vi "GUI_Bella_IP2_plasma1.vi"() -> ()   [LabVIEW 2020]
uses:
  Shared/GUI_Template/GUI_master/tcp_new_data_event.ctl
  Shared/GUI_Template/GUI_master/tcp new data cluster.ctl
panel:
  in  "Position.Axis 2::9":dbl caption="1: Ghost z-position" min=0.0 max=100.0 format="%.3g"
  in  "Position.Axis 1::9":dbl caption="1: Staging Sideview" min=-50.0 max=50.0 format="%.3g"
  in  "GUIdevice 9":string="MCD-PL1-ESP301-1" caption="GUIdevice 4"
  in  "Position.Stage B::19":dbl caption="DPM - Y" min=-100.0 max=105.0 format="%.3g"
  in  "Position.Stage C::18":dbl caption="DPM - Z" min=-100.0 max=100.0 format="%.3g"
  in  "Position.Stage A::18":dbl caption="DPM - X" min=-400.0 max=400.0 format="%.3g"
  in  "GUIdevice 19":string="MCD-PL1-NewmarkDPMY"
  in  "GUIdevice 18":string="MCD-PL1-NewmarkDPMXZ"
  in  "GUIdevice 17":string="IP2-TargetXYZ"
  in  "Position.Axis 1::17":dbl caption="TargetX" min=-200.0 max=200.0 format="%.3g"
  in  "Position.Axis 2::17":dbl caption="Peptide Stage" min=-200.0 max=150.0 format="%.3g"
  in  "Position.Axis 3::17":dbl caption="TargetZ" min=-100.0 max=50.0 format="%.3g"
  in  "GUIdevice 16":string="IP2-TC-ESP5"
  in  "Position.Axis 1::16":dbl caption="Quad 1-2 \n[In = 0, Out = -45]" min=-50.0 max=50.0 format="%.3g"
  in  "Position.Axis 2::16":dbl caption="Quad 3\n[In = 0, Out = 74]" min=-100.0 max=100.0 format="%.3g"
  in  "Position.Axis 3::16":dbl caption="Quad 4 \n[In = 0, Out = 80]" min=-100.0 max=100.0 format="%.3g"
  in  "GUIdevice 15":string="IP2-TC-ESP5"
  in  "Position.Axis 1::15":dbl caption="OPEN" min=-50.0 max=50.0 format="%.3g"
  in  "Position.Axis 2::15":dbl caption="OPEN" min=-100.0 max=100.0 format="%.3g"
  in  "Position.Axis 3::15":dbl caption="OPEN" min=-100.0 max=100.0 format="%.3g"
  in  "GUIdevice 14":string="IP2-TC-ESP3"
  in  "Position.Axis 1::14":dbl caption="TapeDrive Z" min=-25.0 max=25.0 format="%.3g"
  in  "Position.Axis 2::14":dbl caption="IP2-focusdiag-x" min=-25.0 max=25.0 format="%.3g"
  in  "Position.Axis 3::14":dbl caption="Target scatter lens" min=0.0 max=25.0 format="%.3g"
  in  "GUIdevice 13":string="IP2-TC-ESP4"
  in  "Position.Axis 1::13":dbl caption="OAPT-Horz (Yaw)" min=-3.0 max=9.0 format="%.3g"
  in  "Position.Axis 2::13":dbl caption="OAPT-Vert (Pitch)" min=-3.0 max=3.0 format="%.3g"
  in  "Position.Axis 3::13":dbl caption="Profiler Block" min=0.0 max=100.0 format="%.3g"
  in  "GUIdevice 12":string="IP2-BTL-ESP2"
  in  "Position.Axis 1::12":dbl caption="IP2 M5 vrt" min=0.0 max=20.0 format="%.3g"
  in  "Position.Axis 2::12":dbl caption="IP2 M6 (SFL) vrt" min=-20.0 max=20.0 format="%.3g"
  in  "Position.Axis 3::12":dbl caption="IP2 M3 (LFL) vrt" min=-20.0 max=20.0 format="%.3g"
  in  "Position.Axis 3::11":dbl caption="IP2 M3 (LFL) hrz" min=-20.0 max=20.0 format="%.3g"
  in  "Position.Axis 2::11":dbl caption="IP2 M6 (SFL) hrz" min=0.0 max=20.0 format="%.3g"
  in  "Position.Axis 1::11":dbl caption="IP2 M5 hrz" min=-20.0 max=20.0 format="%.3g"
  in  "GUIdevice 11":string="IP2-BTL-ESP1"
  in  "GUIdevice 10":string="IP2-TC-ESP3"
  in  "Position.Axis 2::10":dbl caption="Focus diag X" min=-25.0 max=25.0 format="%.3g"
  in  "Position.Axis 3::8":dbl caption="Focus diag Z" min=-5.0 max=100.0 format="%.3g"
  in  "Position.Axis 2::8":dbl caption="Focus diag Y" min=-5.0 max=150.0 format="%.3g"
  in  "GUIdevice 8":string="IP2-focusdiag-zy" caption="GUIdevice 4"
  out "tcp data event":T1
  in  "stop":bool
  out "error IO 2":errorcluster
  # "Plasma 1 + M Chambers"
  # "TC-ESP3"
  # "TC-ESP4"
  # "TC-ESP5"
  # "TC-ESP6"
  # "Target-XYZ"
  # "BTL-ESP1"
  # "BTL-ESP2"
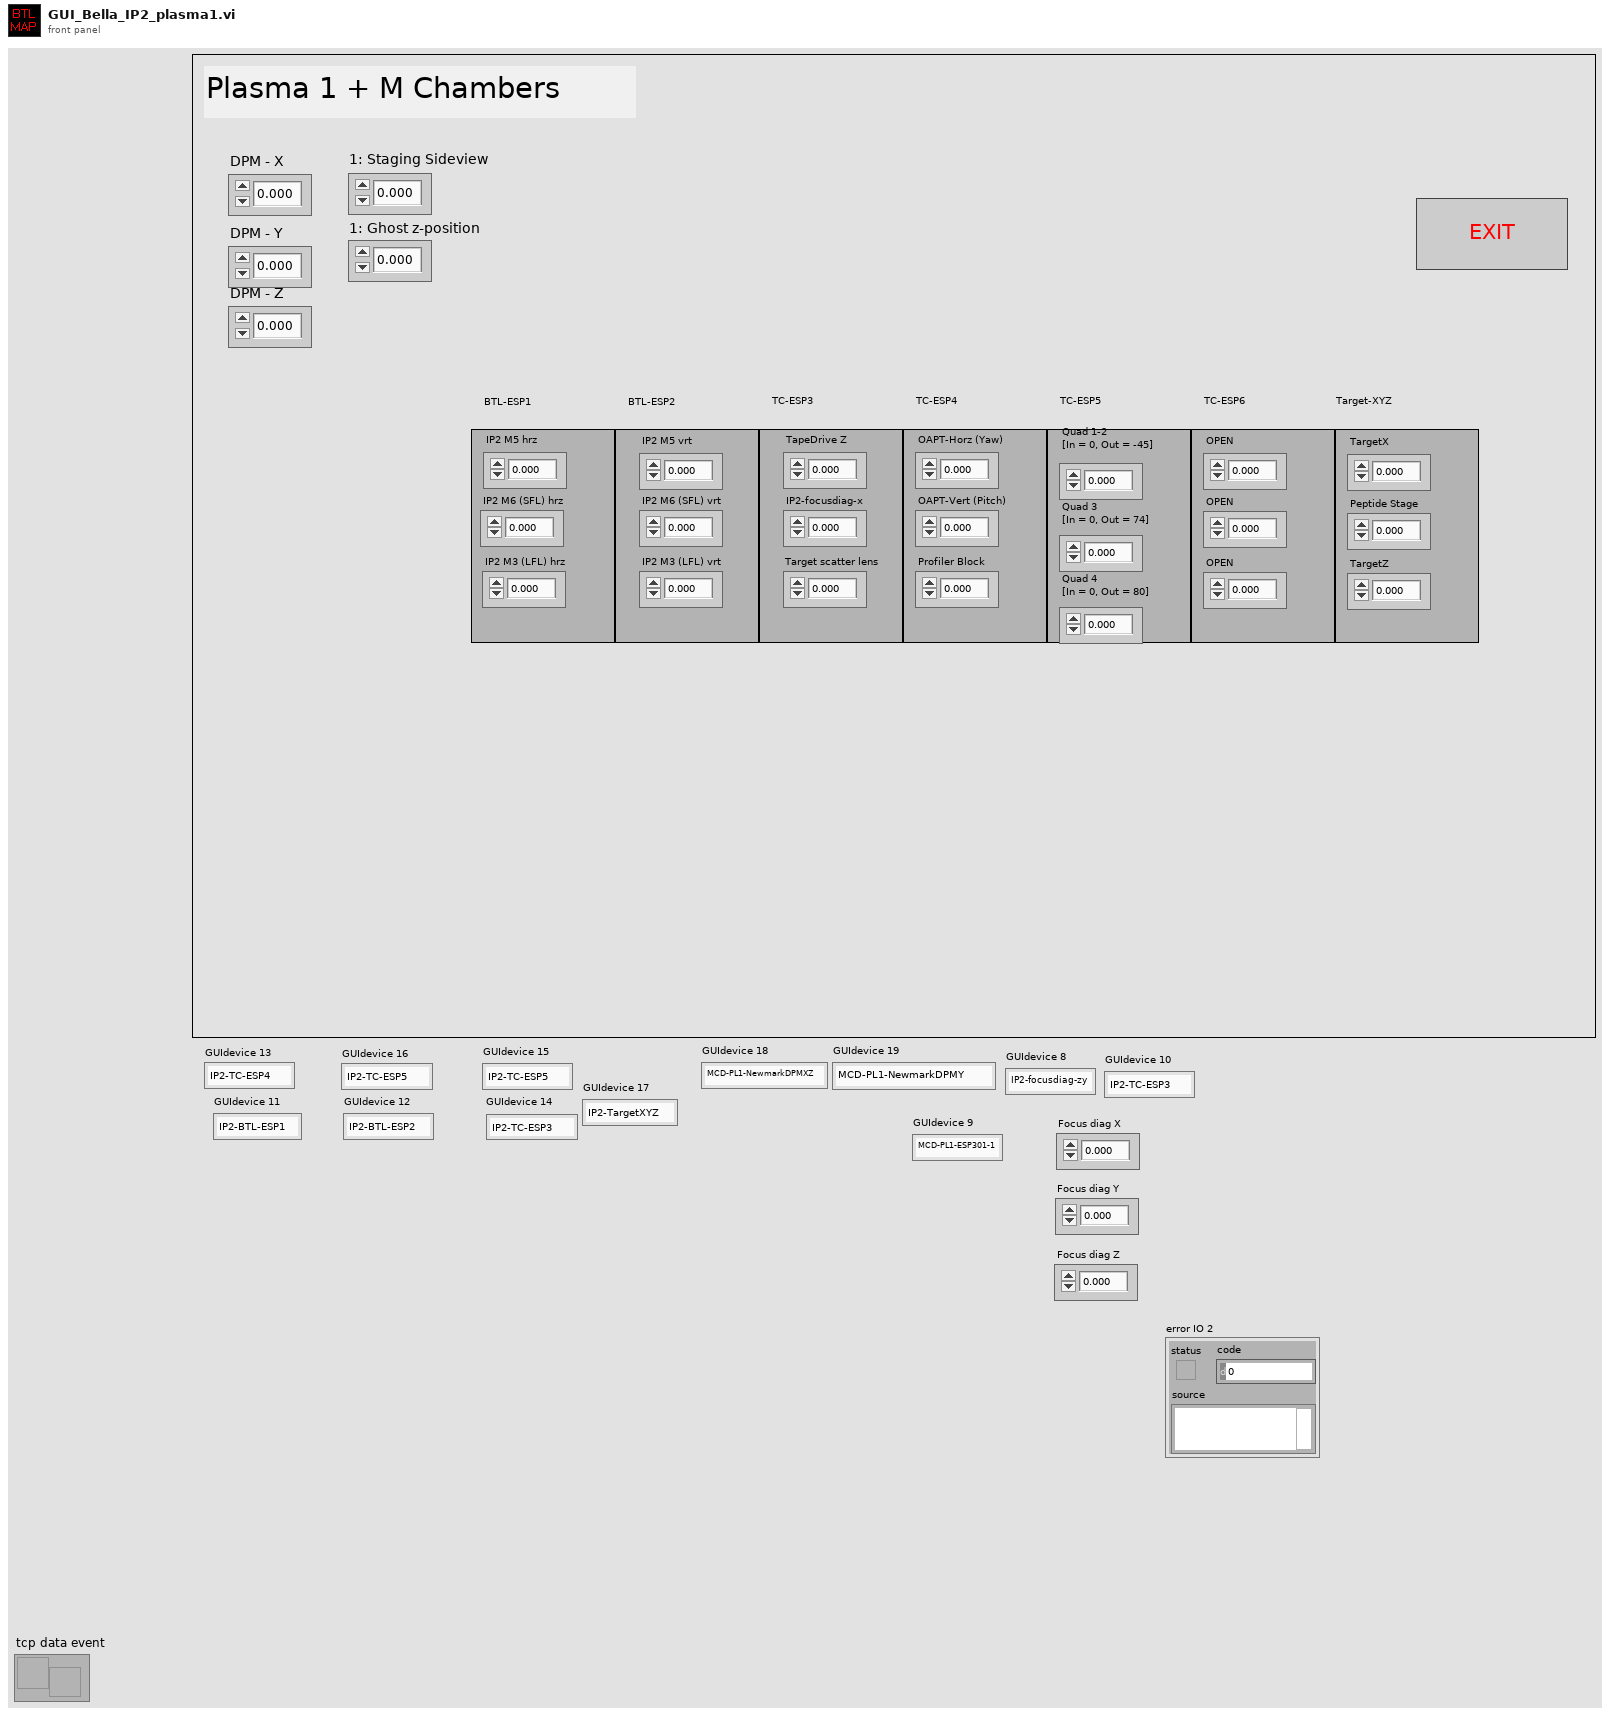
[diagram p1: front panel]
types:
  T1 = typedef "tcp_new_data_event.ctl" = refnum<user-event>
  T2 = typedef "tcp new data cluster.ctl" = cluster{"EventEnum":enum16{"new data", "connection status update"}, "Device name":string}
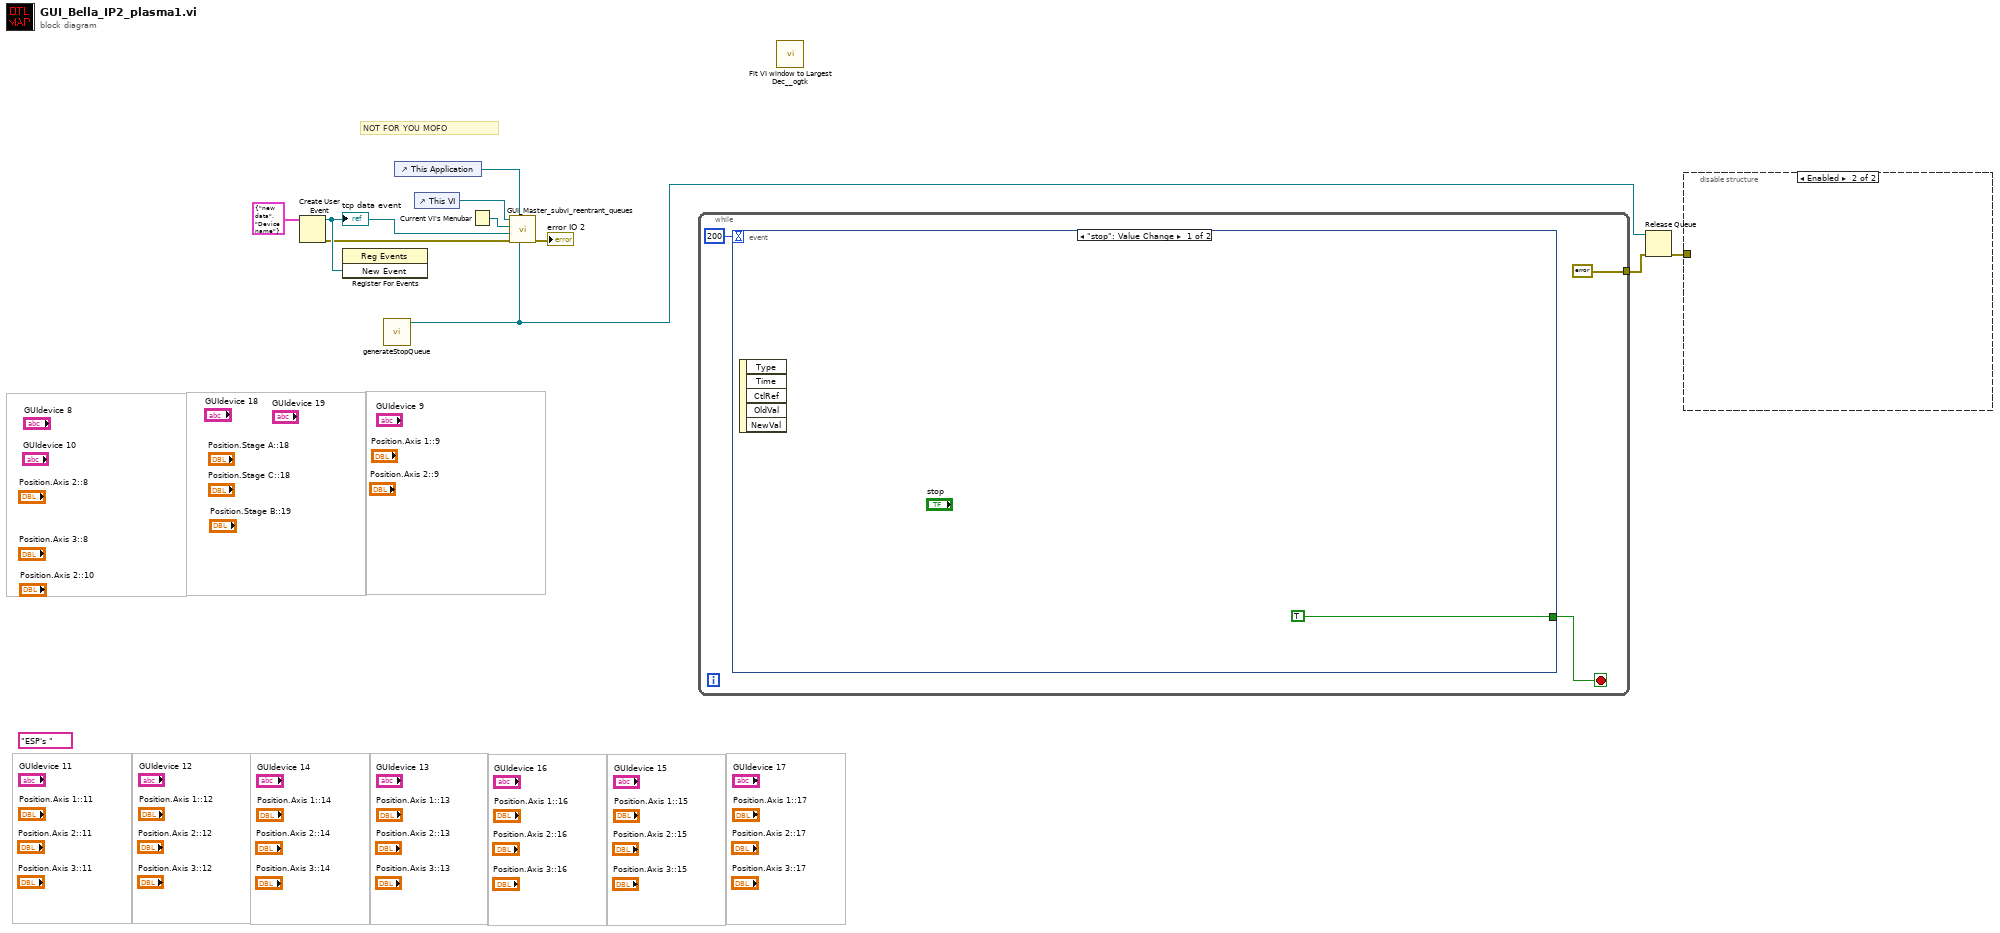
[diagram p0: block diagram]
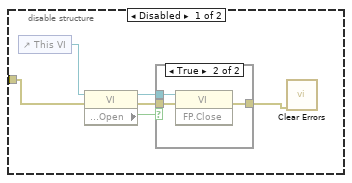
[diagram p2: hidden frame]
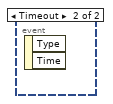
[diagram p4: hidden frame]
diagram:
  (unwired) "ESP's "
  # "NOT FOR YOU MOFO"
  n1 = Create User Event(user event datatype=T2 {"EventEnum"=enum."new data", "Device name"="Device name"} ("New Event")) -> (user event=w9:refnum<user-event>, error out=w8:errorcluster)  [unwired: 1 in]
  "tcp data event" <- w9
  n2 = register-events(w9) -> ()  [unwired: 2 in, 2 out]
  n3 = call "generateStopQueue.vi"() -> ("STOP Queue out"=w3:refnum<queue>)  [unwired: 10 in, 1 out]
  n4 = control-ref of="This Application"() -> (w10:refnum<vi>)
  n5 = control-ref of="This VI"() -> (w5:refnum<vi>)
  n6 = Current VI's Menubar() -> (w6:refnum<k9>)
  n7 = call "GUI_Master_subvi_reentrant_queues.vi"("STOP Queue in"=w3, "This Application"=w10, "error in (no error)"=w8, "tcp data event"=w9, "Caller menu reference"=w6, "Caller VI ref"=w5) -> ("error out"=→"error IO 2":errorcluster)  [unwired: 5 in]
  n8 = while {
    tunnel: [errorcluster {"status"=FALSE, "code"=0, "source"=""} ("error in (no error)")] -> w2
    stop <- w13 stop-if-true
    n9 = event shown="[0] \"stop\": Value Change" {
      selector: _ -> [_ _]
      dyn-events: _ -> [_ _]
      timeout: 200 -> [_ _]
      tunnel: [TRUE ("stop") _] -> w13
      event "stop": Value Change {
        n10 = event-data() -> ()  [unwired: 1 in, 5 out]
      }
      event Timeout {
        n11 = event-data() -> ()  [unwired: 1 in, 2 out]
      }
    }
  }
  n12 = call <userlib>:"Fit VI window to Largest Dec__ogtk.vi"() -> ()  [unwired: 6 in, 2 out]
  n13 = Release Queue(queue=w3, error in (no error)=w2) -> (error out=w1:errorcluster)  [unwired: 1 in, 2 out]
  n14 = disable-structure shown="Enabled" {
    disable-tunnel: w1 -> [w16 _]
    frame Disabled {
      n15 = control-ref of="This VI"() -> (w17:refnum<vi>)
      n16 = property class="VI"(reference=w17, error in=w16) -> (reference out=w19:refnum<vi>, error out=w20:errorcluster, "Front Panel.Open"=w18:bool)
      n17 = case shown="True" w18 {
        tunnel: [w21 w24] -> w15
        tunnel: w20 -> [w21 w23]
        tunnel: w19 -> [_ w22]
        frame False {
        }
        frame True {
          n18 = invoke class="VI" method="FP.Close"(reference=w22, error in=w23) -> (error out=w24:errorcluster)  [unwired: 1 in, 2 out]
        }
      }
      n19 = call <vilib>:"Clear Errors.vi"("error in (no error)"=w15) -> ()  [unwired: 5 in, 2 out]
    }
    frame Enabled {
    }
  }
